vi "BB Reader to Refnum.vi"(3 "BB Reader U64":u64) -> (5 "BB Reader Refnum":T1 {"refnum" format="%.0x"})   [LabVIEW 2021, in "Iceoryx.lvlib"]
uses:
  Iceoryx.lvlib
  Typedef/BB Reader Refnum.ctl
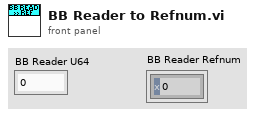
[diagram p1: front panel]
types:
  T1 = typedef "Iceoryx.lvlib/BB Reader Refnum.ctl" = cluster{"refnum":u64, "BB Reader":enum8{"bb_reader"}}
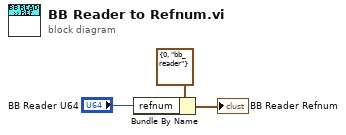
[diagram p0: block diagram]
diagram:
  n1 = Bundle By Name(cluster=T1 {"refnum"=0, "BB Reader"=enum."bb_reader"} ("BB Reader Refnum"), "refnum"="BB Reader U64") -> (→"BB Reader Refnum":T1)
